vi "NetworkUDP_Send.vi"(7 "remote port":u16=5801, 8 "error in (no error)":errorcluster, 9 "timeout ms (25000)":i32=1000, 10 "IP4 Address":u32, 11 "data string":string) -> (0 "error out":errorcluster, 1 "LocalPort":u16, 2 "UDP Network Connection out":refnum<k16>, 3 "Consec Err":i32)   [LabVIEW 2019, in "Trajectory_Library.lvlib"]
doc: "Send a packet of data over the network using the UDP protocol. Data can be directed at a single computer or broadcast to the entire subnet.\n\nInputs:\n -- Remote Port -- UInt16 -- UDP port number to use when sending the data. The reciever must be listening for data on this port number. (Optional. Default: 5801)\n -- Data String -- string -- string of data to be sent. (Generally the maximum reliable size of a UDP packet is approximately 500 bytes. On Ethernet, packets of approximately 1450 bytes may be possible.)\n -- IP4 Address -- UInt32 -- The IP address of the computer listening for this data. If this value is 0, then the data is broadcast to the entire subnet. Use the standard TCP/IP LabVIEW functions to convert a standard IP4 address in the form of 123.123.123.123 to an unsigned integer for this input. (Optional. Default: 0) \n -- Timeout ms -- Int32 -- Timeout value in milliseconds. (Optional. Default: 1000 )\n -- Error in -- Error cluster -- Propagated error cluster. (Optional. Default: no error)\n\nOutputs:\n -- Consec Err -- Int32 -- Counter indicating the number of consecutive errors that have occured.\n -- UDP Network Connection -- UDP Connection Reference -- Reference to the UDP network connection. When finished with communication, the connection should be closed.\n -- Error out -- Error cluster -- Current propagated error cluster."
uses:
  Trajectory_Library.lvlib
panel:
  # "UDP WRITE"
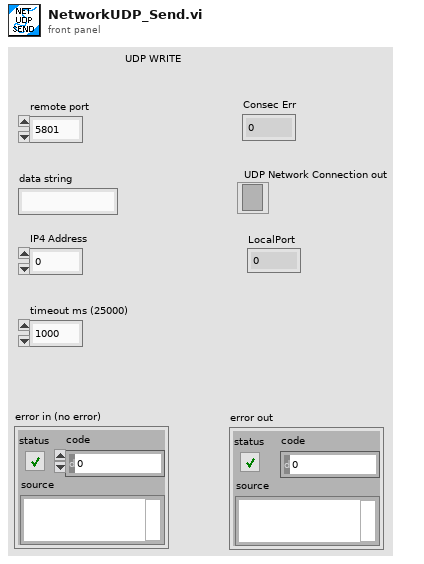
[diagram p1: front panel]
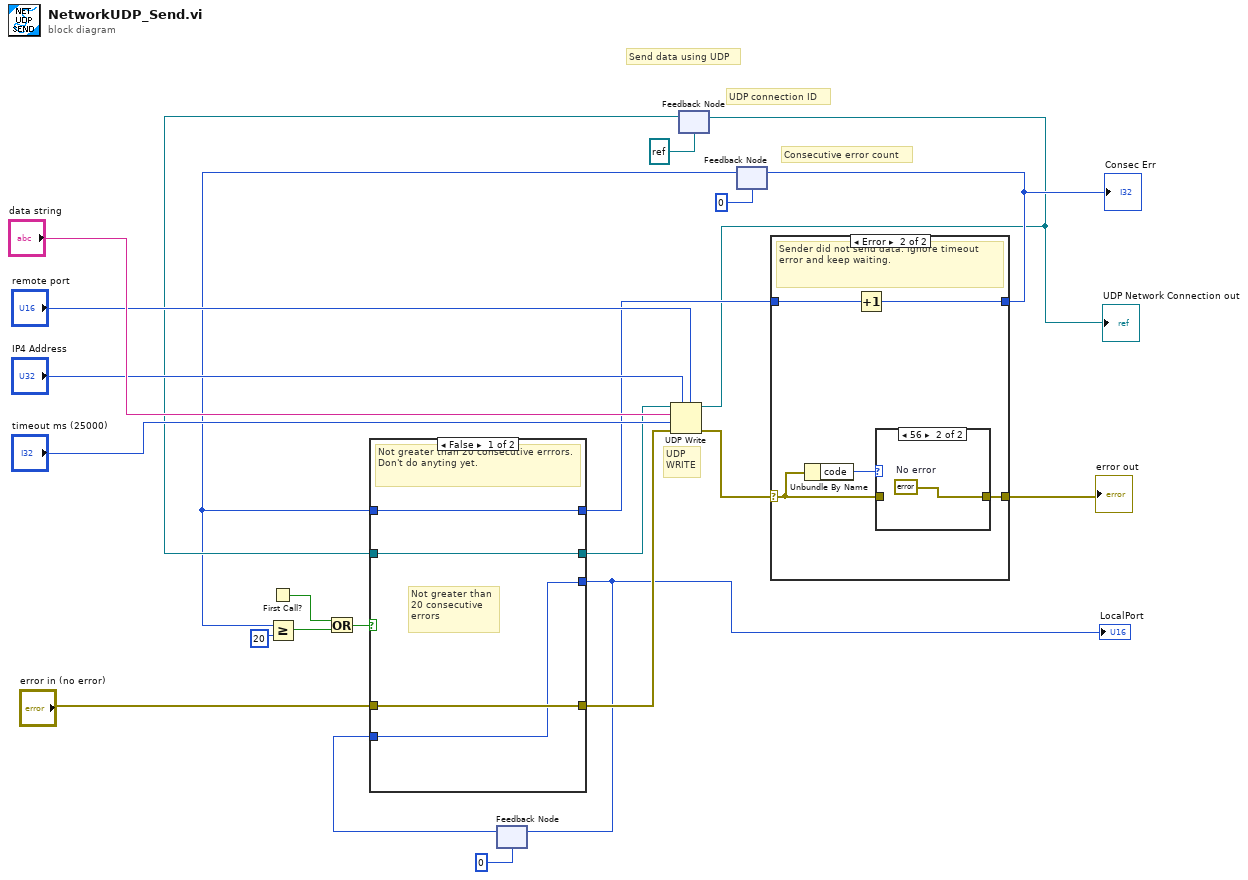
[diagram p0: block diagram]
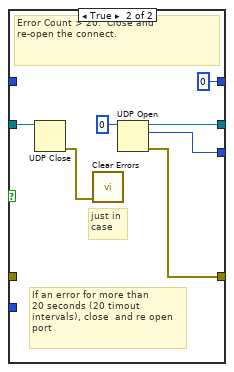
[diagram p2: hidden frame]
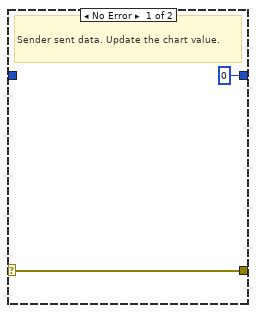
[diagram p3: hidden frame]
diagram:
  # "Send data using UDP"
  # "UDP connection ID"
  # "Consecutive error count"
  # "UDP\nWRITE"
  n1 = First Call?() -> (First Call?: T/F=w6:bool)
  n2 = feedback #1(u16 0 ("service name")) -> (w1:u16)
  n3 = feedback #2(refnum<k16> refnum ("port")) -> (w16:refnum<k16>)
  n4 = feedback #3(0) -> (w5:i32)
  n5 = Greater Or Equal?(x=w5, y=20) -> (x >= y?=w4:bool)
  n6 = Or(x=w6, y=w4) -> (x .or. y?=w7:bool)
  n7 = case shown="False" w7 {
    tunnel: w5 -> [w27 _]
    tunnel: [w27 0] -> w15
    tunnel: w16 -> [w26 w34]
    tunnel: [w26 w33] -> w14
    tunnel: "error in (no error)" -> [w25 _]
    tunnel: [w25 w32] -> w13
    tunnel: [w24 w28] -> w3
    tunnel: w1 -> [w24 _]
    frame False {
      # "Not greater than\n20 consecutive\nerrors"
      # "Not greater than 20 consecutive errrors.  Don't do anyting yet."
    }
    frame True {
      # "just in \ncase"
      # "If an error for more than\n20 seconds (20 timout\nintervals), close  and re open \nport"
      # "Error Count > 20.  Close and \nre-open the connect."
      n8 = UDP Close(connection ID=w34) -> (error out=w29:errorcluster)  [unwired: 1 in, 1 out]
      n9 = call <vilib>:"Clear Errors.vi"("error in (no error)"=w29) -> ()  [unwired: 5 in, 2 out]
      n10 = UDP Open(11:u16 0 ("port")) -> (port=w33:refnum<k16>, 0:w32:errorcluster, 2:w28:u16)  [unwired: 4 in]
    }
  }
  "LocalPort" <- w3
  n11 = feedback-in #1(w3) -> ()
  n12 = UDP Write(address="IP4 Address", port or service name="remote port", connection ID=w14, data in="data string", 8:w13, 9:"timeout ms (25000)") -> (error out=w17:errorcluster, 3:w10:refnum<k16>)
  "UDP Network Connection out" <- w10
  n13 = feedback-in #2(w10) -> ()
  n14 = case shown="Error" w17 {
    selector: w17 -> [w36 w40]
    tunnel: [w36 w39] -> w9
    tunnel: w15 -> [_ w38]
    tunnel: [0 w37] -> w11
    frame No Error {
      (unwired) 0
      # "Sender sent data. Update the chart value."
    }
    frame Error {
      # "Sender did not send data. Ignore timeout error and keep waiting."
      n15 = Unbundle By Name(w40) -> ("code"=w41:i32)
      n16 = Increment(x=w38) -> (x+1=w37:i32)
      n17 = case shown="56" w41 {
        tunnel: w40 -> [w42 _]
        tunnel: [w42 w43] -> w39
        frame Default {
        }
        frame 56 {
          w43 = errorcluster {"status"=FALSE, "code"=0, "source"=""}  # No error
        }
      }
    }
  }
  "Consec Err" <- w11
  "error out" <- w9
  n18 = feedback-in #3(w11) -> ()
